vi "Init.vi"(8 "error in (no error)":errorcluster, 11 "TCP Text Writer in":refnum<class "TCP Text Writer.lvclass">) -> (0 "error out":errorcluster, 3 "TCP Text Writer out":refnum<class "TCP Text Writer.lvclass">)   [LabVIEW 2020, in "TALOS.lvlib" / "TCP Text Writer.lvlib" / "TCP Text Writer.lvclass"]
uses:
  TCP Text Writer.lvclass
  C:/LabVIEW Code/TALOS/talos/Internal uServices/System uServices/TCP Writer/TCP Writer/TCP Writer.lvclass
  TCP Text Writer.lvclass/TCP Text Writer.ctl
  TCP Writer/TCP Writer/TCP Writer.lvclass
  Father of all uServices/Father of all uServices/Father of all uServices.lvclass
  C:/LabVIEW Code/TALOS/talos/Father of all uServices/Father of all uServices/Father of all uServices.lvclass
  C:/LabVIEW Code/TALOS/talos/Ancestor/Ancestor/Ancestor.lvclass
  C:/LabVIEW Code/TALOS/builds/Actor Framework PPL/Actor Framework.lvlibp/1abvi3w/vi.lib/ActorFramework/Actor/Actor.lvclass
  C:/LabVIEW Code/TALOS/talos/Internal uServices/System uServices/TCP Text Writer/TCP Text Writer.lvclass
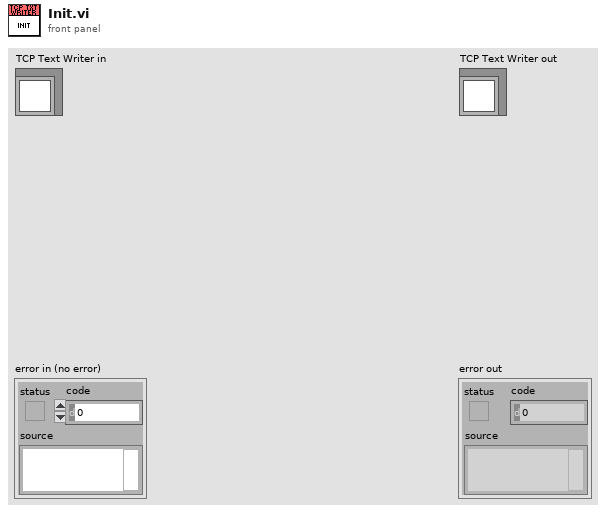
[diagram p1: front panel]
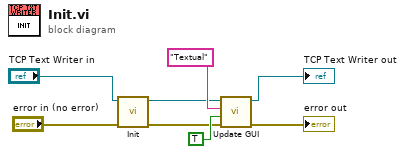
[diagram p0: block diagram]
diagram:
  n1 = call-parent "Init.vi"("error in (no error)"="error in (no error)", "TCP Writer in"="TCP Text Writer in") -> ("error out"=w3:errorcluster, "TCP Writer out"=w4:refnum<class "TCP Text Writer.lvclass">)  [unwired: 8 in]
  n2 = call "Update GUI.vi"("error in (no error)"=w3, "Data"=TRUE ("Textual"), "GUI Item Name"="Textual", "uService Template in"=w4) -> ("error out"=→"error out":errorcluster, "uService Template out"=→"TCP Text Writer out":refnum<class "TCP Text Writer.lvclass">)  [unwired: 6 in]
